vi "PeriodicDBsave.vi"(6 "Check pace (sec)":dbl=5.0, 8 "error in (no error)":errorcluster, 11 "FAMM in":refnum<class "FAMM.lvclass">) -> (0 "error out":errorcluster, 3 "FAMM out":refnum<class "FAMM.lvclass">)   [LabVIEW 2020, in "Sgraph_lib_V1.lvlib" / "FAMM.lvclass"]
doc: "Andre Koelewijn\nRev 2\n30 jun 2021\n\nPeriodic check if data has to be saved to the database,\nthe pace input defines the inteval at which the data memory is saved.\n\nData is saved by the DBAL Service (to prevent FAMM latency)"
uses:
  FAMM.lvclass
  DBAL/controls/DBAL_Command.ctl
  DBAL/controls/DBAL-commands.ctl
  FAMM.lvclass/FAMM.ctl
  DBAL/DBAL.lvclass
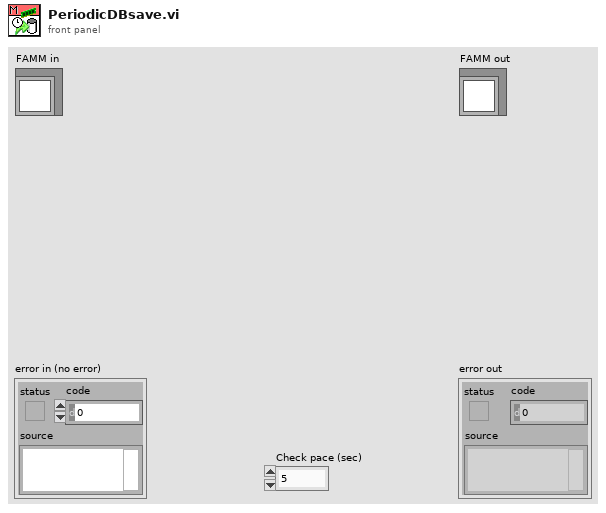
[diagram p1: front panel]
types:
  T1 = typedef "Sgraph_lib_V1.lvlib/DBAL.lvclass/DBAL-commands.ctl" = enum16{"idle", "SavePAQdata", "ExitService"}
  T2 = typedef "Sgraph_lib_V1.lvlib/DBAL.lvclass/DBAL_Command.ctl" = cluster{"Source":string, "Command":T1, "Time Stamp":timestamp, "data":variant}
  T3 = cluster{"TableName":string, "Data2save":cluster{"TAGs":string[], "time":dbl[], "TagsData":cluster{"data":dbl[], "max":dbl[], "min":dbl[], "status":u32[]}[]}}[]
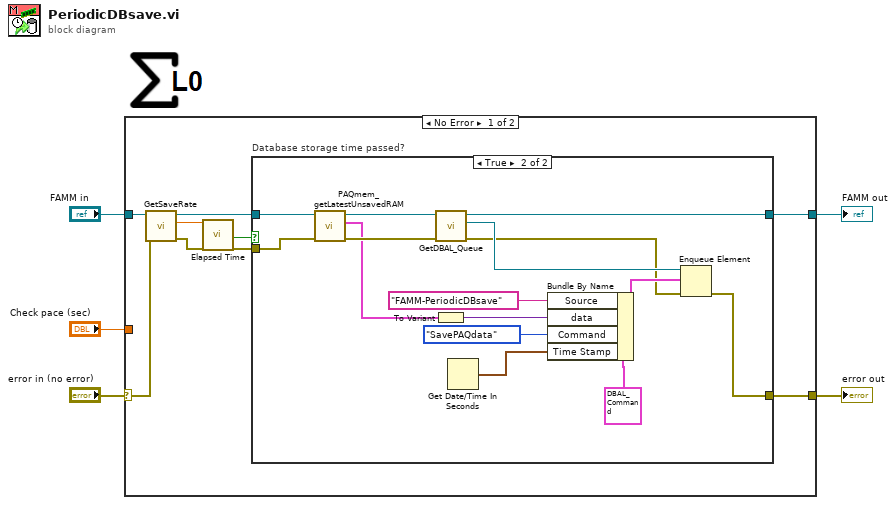
[diagram p0: block diagram]
diagram:
  n1 = case shown="No Error" "error in (no error)" {
    selector: "error in (no error)" -> [w8 w33]
    tunnel: [w11 w33] -> w4
    tunnel: [w13 w32] -> w2
    tunnel: "FAMM in" -> [w9 w32]
    tunnel: "Check pace (sec)" -> [_ _]
    frame No Error {
      n2 = call "GetSaveRate.vi"("error in (no error)"=w8, "FAMM in"=w9) -> ("error out"=w7:errorcluster, "Dbase saving period (sec)"=w6:dbl, "FAMM out"=w10:refnum<class "FAMM.lvclass">)  [unwired: 7 in]
      n3 = call "Elapsed Time"("Time Target (s)"=w6, "error in (no error)"=w7) -> ("Time has Elapsed"=w14:bool, "error out"=w12:errorcluster)  [unwired: 10 in, 6 out]
      n4 = case "Database storage time passed?" shown="True" w14 {
        tunnel: w10 -> [w16 w31]
        tunnel: [w16 w28] -> w13
        tunnel: w12 -> [w15 w30]
        tunnel: [w15 w17] -> w11
        frame False {
        }
        frame True {
          n5 = call "PAQmem_getLatestUnsavedRAM.vi"("error in (no error)"=w30, "FAMM in"=w31) -> ("error out"=w27:errorcluster, "Data_2_Save"=w24:T3, "FAMM out"=w29:refnum<class "FAMM.lvclass">)  [unwired: 7 in]
          n6 = call "GetDBAL_Queue.vi"("error in (no error)"=w27, "FAMM in"=w29) -> ("error out"=w18:errorcluster, "DBAL-Queue"=w26:refnum<queue>, "FAMM out"=w28:refnum<class "FAMM.lvclass">)  [unwired: 7 in]
          n7 = To Variant(anything=w24) -> (Variant=w23:variant)
          n8 = Get Date/Time In Seconds() -> (seconds since 1Jan1904=w20:timestamp)
          n9 = Bundle By Name(cluster=T2 {"Source"="", "Command"=enum."idle", "Time Stamp"=timestamp(0 s since 1904-01-01), "data"=variant} ("element"), "Source"="FAMM-PeriodicDBsave", "data"=w23, "Command"=DBAL-commands."SavePAQdata", "Time Stamp"=w20) -> (w19:T2)
          n10 = Enqueue Element(queue=w26, element=w19, error in (no error)=w18) -> (error out=w17:errorcluster)  [unwired: 1 in, 2 out]
        }
      }
    }
    frame Error {
    }
  }
  "error out" <- w4
  "FAMM out" <- w2
